vi "Discretization_DiscretizeR.vi"(6 "dT_Seconds":dbl, 9 "ContR":T1, 11 "Outputs":i32) -> (0 "Size Coerced":bool, 3 "DiscR":T1)   [LabVIEW 2019, in "Trajectory_Library.lvlib"]
doc: "Returns a discretized version of the provided continuous measurement noise covariance matrix. Note that dt=0.0 divides R by zero.\n \nInputs:\n - Outputs -- the number of outputs.\n - R -- Continuous measurement noise covariance matrix.\n - dtSeconds -- Discretization timestep.\n\nOutputs:\n - DiscR -- Discretized version of the provided continuous measurement noise covariance matrix.\n - SizeCoerced -- If TRUE, an error occured."
uses:
  Trajectory_Library.lvlib
  <vilib>/Analysis/Matrix/Datatypes/RealMatrix.ctl
  <vilib>/Analysis/Matrix/NI_Matrix.lvlib
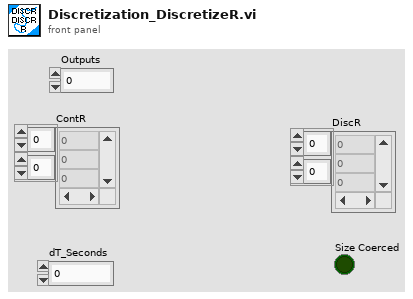
[diagram p1: front panel]
types:
  T1 = typedef "NI_Matrix.lvlib/RealMatrix.ctl" = dbl[][]
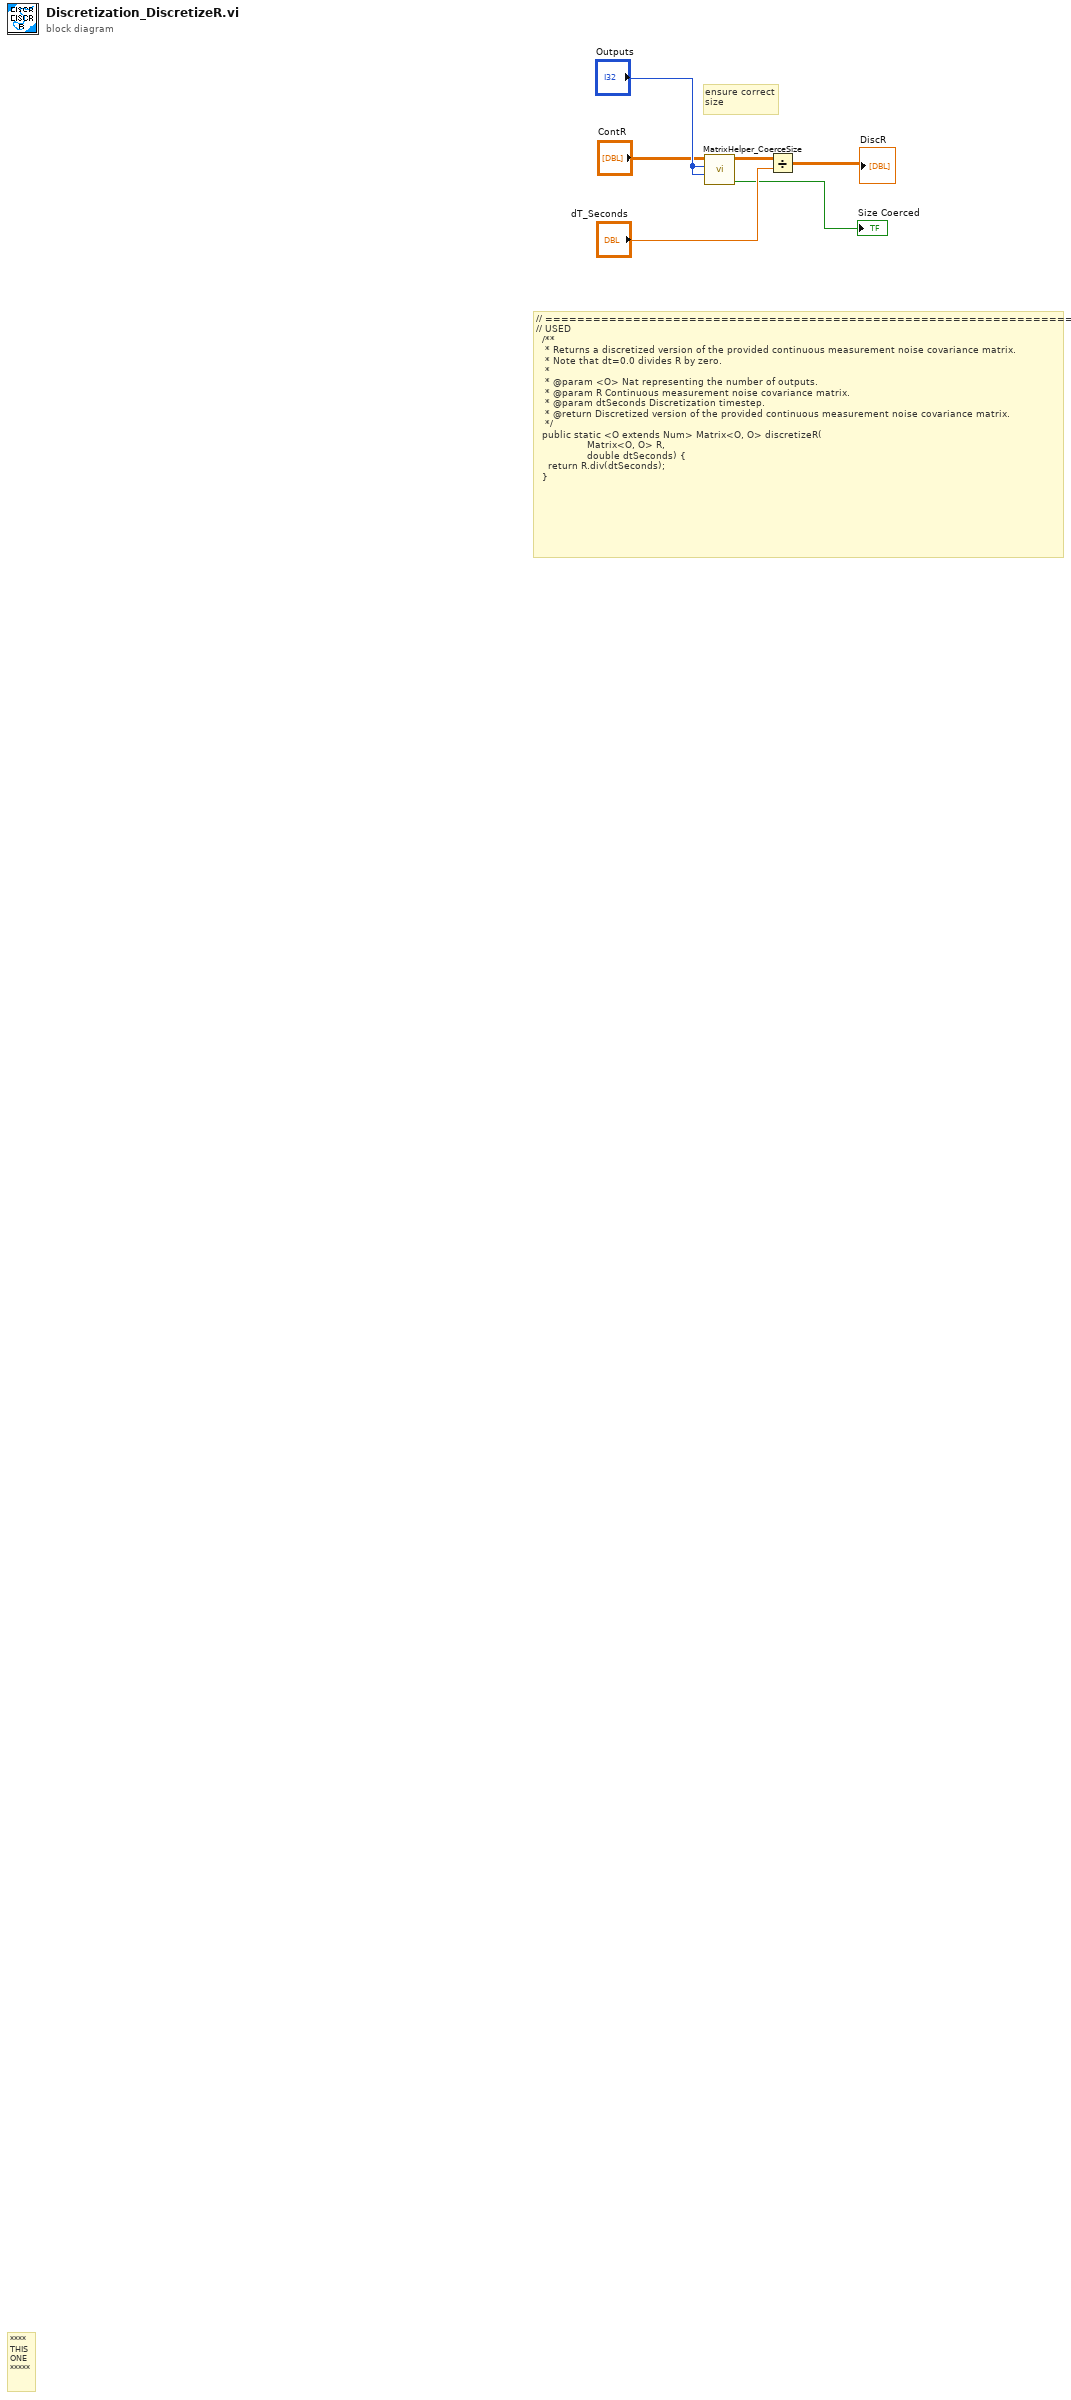
[diagram p0: block diagram]
diagram:
  # "// ==================================================================\n// USED\n  /**\n   * Returns a discretized version of the provided continuous measurement noise covariance matrix.\n   * Note that dt=0.0 divides R by zero.\n   *\n   * @param <O> Nat representing the number of outputs.\n   * @param R Continuous measurement noise covariance matrix.\n   * @param dtSeconds Discretization timestep.\n   * @return Discretized version of the provided continuous measurement noise covariance matrix.\n   */\n  public static <O extends Num> Matrix<O, O> discretizeR(\n                 Matrix<O, O> R, \n                 double dtSeconds) {\n    return R.div(dtSeconds);\n  }"
  # "ensure correct\nsize"
  # "****\nTHIS\nONE\n*****"
  n1 = call "MatrixHelper_CoerceSize.vi"("Columns"="Outputs", "Rows"="Outputs", "input matrix"="ContR") -> ("Coerced"=→"Size Coerced":bool, "output matrix"=w2:T1)  [unwired: 7 in]
  n2 = Divide(x=w2, y="dT_Seconds") -> (x/y=→"DiscR":T1)
